vi "MP3 Parse Frames.vi"(0 "File Data":u8[](array[numeric])) -> (4 "Main Data":u8[](array[numeric]), 6 "Frames":i32[](array[numeric]), 8 "Frame Count":i32)   [LabVIEW 2026]
doc: "Splits an MP3 file into its frames (MPEG-1 Layer III only) and joins all main data into one stream.\nAn ID3v2 tag at the start is skipped. At each position the 32-bit header is checked (sync 0x7FF, MPEG-1, Layer III, valid bitrate and sample rate); anything else advances one byte, which also resynchronises after damage. A Xing/Info frame (VBR header) is skipped.\nFrames is a flat array, 51 values per frame: sample-rate index, mode, mode extension, channels, the bit position in Main Data where this frame's main data starts (main_data_begin points back into earlier frames - the bit reservoir), then the 46 side-information fields (24 for mono, zero padded).\nMain Data has 4 zero bytes appended so bit reads near the end stay in range."
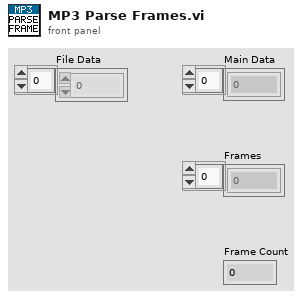
[diagram p1: front panel]
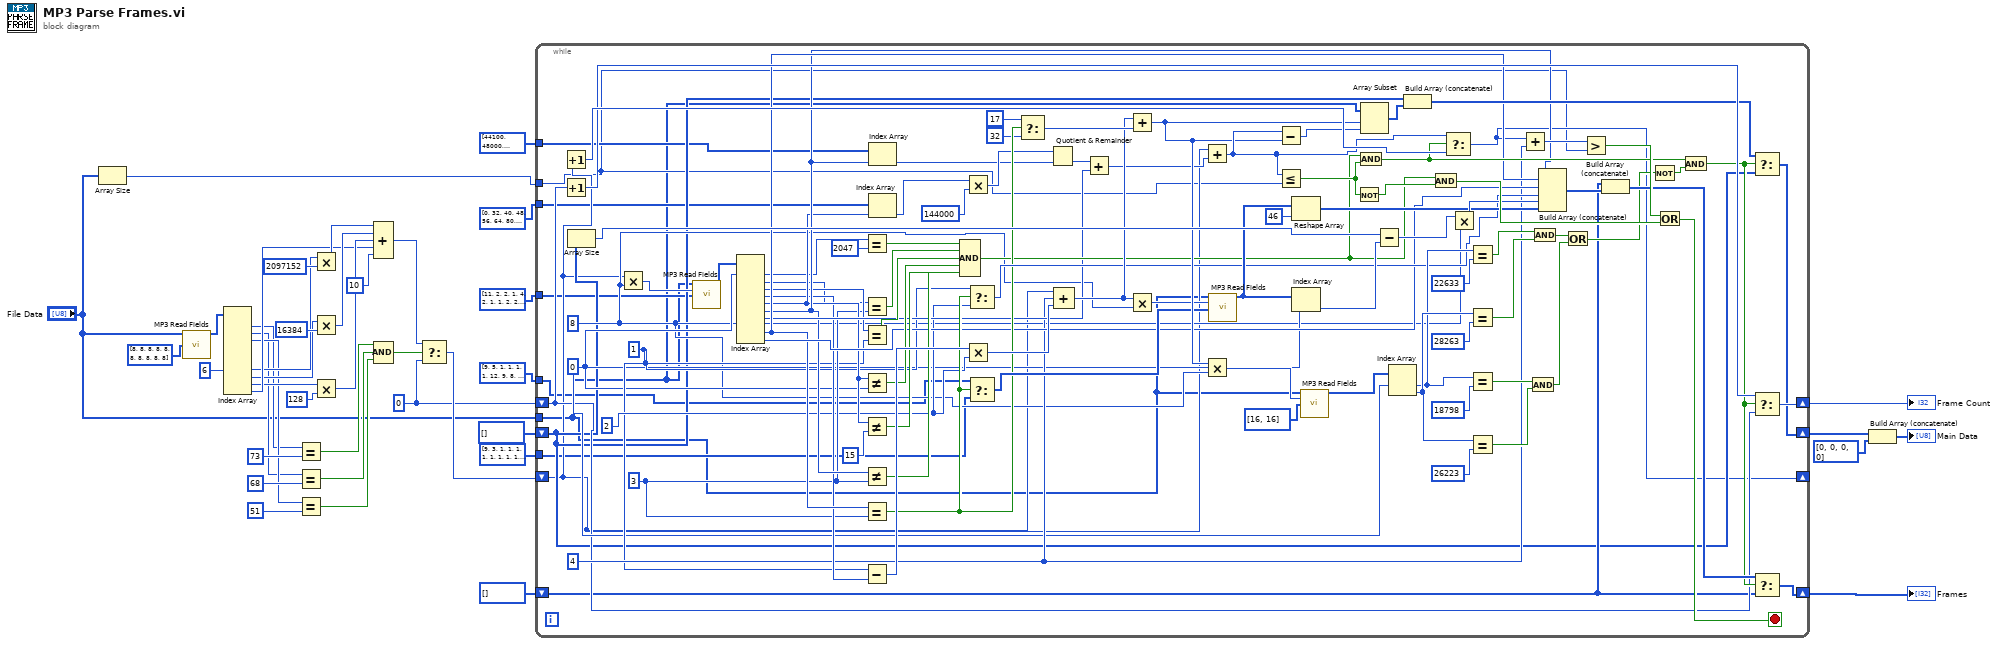
[diagram p0: block diagram]
diagram:
  w4 = 0
  n1 = Array Size(array="File Data") -> (size(s)=w29:i32)
  n2 = call "MP3 Read Fields.vi"("Data"="File Data", "Widths"=i32[] [8, 8, 8, 8, 8, 8, 8, 8, 8, 8]) -> ("Fields"=w5:i32[])  [unwired: 12 in, 1 out]
  n3 = Index Array(array=w5, index #7=6 ("index")) -> (element #1=w6:i32, element #2=w7:i32, element #3=w8:i32, element #7=w9:i32, element #8=w10:i32, element #9=w11:i32, element #10=w12:i32)  [unwired: 9 in, 3 out]
  n4 = Equal?(x=w6, y=73) -> (x = y?=w16:bool)
  n5 = Equal?(x=w7, y=68) -> (x = y?=w17:bool)
  n6 = Equal?(x=w8, y=51) -> (x = y?=w18:bool)
  n7 = Multiply(x=w9, y=2097152) -> (x*y=w23:i32)
  n8 = Multiply(x=w10, y=16384) -> (x*y=w24:i32)
  n9 = Multiply(x=w11, y=128) -> (x*y=w25:i32)
  n10 = Compound Arithmetic op=ADD(w23, w24, w25, w12, 10) -> (w27:i32)
  n11 = Compound Arithmetic op=AND(w16, w17, w18) -> (w19:bool)
  n12 = Select(t=w27, s=w19, f=w4) -> (s? t:f=w28:i32)
  n13 = while {
    tunnel: "File Data" -> [w42]
    tunnel: i32[] [11, 2, 2, 1, 4, 2, 1, 1, 2, 2, 1, 1, 2] -> [w44]
    tunnel: i32[] [9, 5, 1, 1, 1, 1, 12, 9, 8, 4, 1, 22, 1, 1, 1, 12, 9, 8, 4, 1, 22, 1, 1, 1] -> [w45]
    tunnel: i32[] [9, 3, 1, 1, 1, 1, 1, 1, 1, 1, 12, 9, 8, 4, 1, 22, 1, 1, 1, 12, 9, 8, 4, 1, 22, 1, 1, 1, 12, 9, 8, 4, 1, 22, 1, 1, 1, 12, 9, 8, 4, 1, 22, 1, 1, 1] -> [w46]
    tunnel: i32[] [0, 32, 40, 48, 56, 64, 80, 96, 112, 128, 160, 192, 224, 256, 320, 0] -> [w47]
    tunnel: i32[] [44100, 48000, 32000, 0] -> [w48]
    shift-right: [w52] -> w37
    shift-left: u8[] [] -> [w51]
    shift-right: [w54] -> w38
    shift-left: i32[] [] -> [w53]
    shift-right: [w56] -> w39
    shift-left: w4 -> [w55]
    tunnel: w29 -> [w43]
    shift-right: [w50] -> _
    shift-left: w28 -> [w49]
    stop <- w139 stop-if-true
    w62 = 4
    w61 = 3
    w60 = 2
    w59 = 1
    w58 = 0
    w57 = 8
    n14 = Increment(x=w49) -> (x+1=w134:i32)
    n15 = Increment(x=w55) -> (x+1=w133:i32)
    n16 = Array Size(array=w51) -> (size(s)=w127:i32)
    n17 = Multiply(x=w49, y=w57) -> (x*y=w74:i32)
    n18 = call "MP3 Read Fields.vi"("Data"=w42, "Bit Position"=w74, "Widths"=w44) -> ("Fields"=w75:i32[])  [unwired: 11 in, 1 out]
    n19 = Index Array(array=w75, index #1=w58) -> (element #1=w76:i32, element #2=w77:i32, element #3=w78:i32, element #4=w79:i32, element #5=w80:i32, element #6=w81:i32, element #7=w82:i32, element #9=w83:i32, element #10=w84:i32)  [unwired: 9 in, 1 out]
    n20 = Equal?(x=w76, y=2047) -> (x = y?=w85:bool)
    n21 = Equal?(x=w77, y=w61) -> (x = y?=w86:bool)
    n22 = Equal?(x=w78, y=w59) -> (x = y?=w87:bool)
    n23 = Not Equal?(x=w80, y=w58) -> (x != y?=w88:bool)
    n24 = Not Equal?(x=w80, y=15) -> (x != y?=w89:bool)
    n25 = Not Equal?(x=w81, y=w61) -> (x != y?=w90:bool)
    n26 = Equal?(x=w83, y=w61) -> (x = y?=w97:bool)
    n27 = Subtract(x=w59, y=w79) -> (x-y=w99:i32)
    n28 = Index Array(array=w48, index=w81) -> (element=w93:i32)
    n29 = Index Array(array=w47, index=w80) -> (element=w92:i32)
    n30 = Compound Arithmetic op=AND(w85, w86, w87, w88, w89, w90) -> (w91:bool)
    n31 = Multiply(x=w92, y=144000) -> (x*y=w94:i32)
    n32 = Multiply(x=w99, y=w60) -> (x*y=w100:i32)
    n33 = Select(t=w59, s=w97, f=w60) -> (s? t:f=w98:i32)
    n34 = Select(t=w45, s=w97, f=w46) -> (s? t:f=w103:i32[])
    n35 = Select(t=17, s=w97, f=32) -> (s? t:f=w102:i32)
    n36 = Quotient & Remainder(x=w94, y=w93) -> (floor(x/y)=w95:i32)  [unwired: 1 out]
    n37 = Compound Arithmetic op=ADD(w49, w62, w100) -> (w101:i32)
    n38 = Add(x=w95, y=w82) -> (x+y=w96:i32)
    n39 = Add(x=w101, y=w102) -> (x+y=w107:i32)
    n40 = Multiply(x=w101, y=w57) -> (x*y=w104:i32)
    n41 = Add(x=w49, y=w96) -> (x+y=w108:i32)
    n42 = Multiply(x=w107, y=w57) -> (x*y=w111:i32)
    n43 = call "MP3 Read Fields.vi"("Data"=w42, "Bit Position"=w104, "Widths"=w103) -> ("Fields"=w105:i32[])  [unwired: 11 in, 1 out]
    n44 = Subtract(x=w108, y=w107) -> (x-y=w109:i32)
    n45 = Less Or Equal?(x=w108, y=w43) -> (x <= y?=w122:bool)
    n46 = Reshape Array(w105, 46) -> (w106:i32[])
    n47 = Index Array(array=w105, index=w58) -> (element=w126:i32)
    n48 = call "MP3 Read Fields.vi"("Data"=w42, "Bit Position"=w111, "Widths"=i32[] [16, 16]) -> ("Fields"=w112:i32[])  [unwired: 11 in, 1 out]
    n49 = Not(x=w122) -> (.not. x?=w137:bool)
    n50 = And(x=w91, y=w122) -> (x .and. y?=w123:bool)
    n51 = Array Subset(array=w42, index=w107, length=w109) -> (w110:u8[])
    n52 = Subtract(x=w127, y=w126) -> (x-y=w128:i32)
    n53 = Index Array(array=w112, index #1=w58) -> (element #1=w113:i32, element #2=w114:i32)  [unwired: 1 in]
    n54 = Build Array (concatenate)(w51, w110) -> (w131:u8[])
    n55 = And(x=w91, y=w137) -> (x .and. y?=w138:bool)
    n56 = Select(t=w108, s=w123, f=w134) -> (s? t:f=w50:i32)
    n57 = Multiply(x=w128, y=w57) -> (x*y=w129:i32)
    n58 = Equal?(x=w113, y=22633) -> (x = y?=w115:bool)
    n59 = Equal?(x=w114, y=28263) -> (x = y?=w116:bool)
    n60 = Equal?(x=w113, y=18798) -> (x = y?=w117:bool)
    n61 = Equal?(x=w114, y=26223) -> (x = y?=w118:bool)
    n62 = Add(x=w50, y=w62) -> (x+y=w135:i32)
    n63 = And(x=w117, y=w118) -> (x .and. y?=w120:bool)
    n64 = And(x=w115, y=w116) -> (x .and. y?=w119:bool)
    n65 = Build Array (concatenate)(w81, w83, w84, w98, w129, w106) -> (w130:i32[])
    n66 = Or(x=w119, y=w120) -> (x .or. y?=w121:bool)
    n67 = Greater?(x=w135, y=w43) -> (0:w136:bool)
    n68 = Build Array (concatenate)(w53, w130) -> (w132:i32[])
    n69 = Not(x=w121) -> (.not. x?=w124:bool)
    n70 = Or(x=w136, y=w138) -> (x .or. y?=w139:bool)
    n71 = And(x=w123, y=w124) -> (x .and. y?=w125:bool)
    n72 = Select(t=w131, s=w125, f=w51) -> (s? t:f=w52:u8[])
    n73 = Select(t=w133, s=w125, f=w55) -> (s? t:f=w56:i32)
    n74 = Select(t=w132, s=w125, f=w53) -> (s? t:f=w54:i32[])
  }
  "Frames" <- w38
  "Frame Count" <- w39
  n75 = Build Array (concatenate)(w37, u8[] [0, 0, 0, 0]) -> (→"Main Data":u8[])
